vi "XPN Get Sensor Info.vi"(7 "height":i32, 8 "error in (no error)":errorcluster, 9 "width":i32, 10 "snSize":i32, 11 "serialNumber":string) -> (0 "error out":errorcluster, 1 "width out":i32, 2 "function return":i32, 3 "serialNumber out":string, 5 "height out":i32)   [LabVIEW 2022 SP3, in "xPanelWrapper.lvlib"]
doc: "XPN_API int XPN_GetSensorInfo(char* serialNumber, int snSize,\n int* width, int* height);"
uses:
  xPanelWrapper.lvlib
  xPanelWrapper.dll
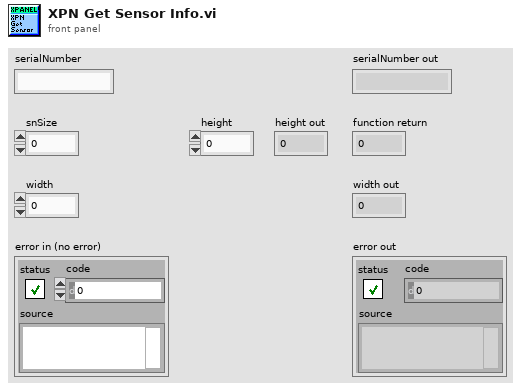
[diagram p1: front panel]
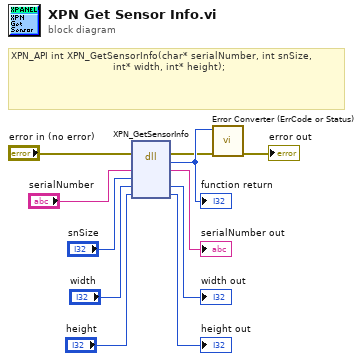
[diagram p0: block diagram]
diagram:
  # "XPN_API int XPN_GetSensorInfo(char* serialNumber, int snSize,\n                                  int* width, int* height);"
  n1 = dll-call lib="E:/SourceCodes/image-harvest/ImageHandler/xPanelWrapperLvLib/xPanelWrapper.*" fn="XPN_GetSensorInfo"(error in="error in (no error)", "serialNumber"="serialNumber", "snSize"="snSize", "width"="width", "height"="height") -> (error out=w2:errorcluster, w11:i32, "serialNumber"=→"serialNumber out":string, "width"=→"width out":i32, "height"=→"height out":i32)  [unwired: 3 in, 1 out]
  "function return" <- w11
  n2 = call "Error Converter (ErrCode or Status).vi"("error in (no error)"=w2, "error code"=w11) -> ("error out"=→"error out":errorcluster)  [unwired: 9 in]
